vi "Test Client Timeout Returns Error.vi"(8 "error in (no error)":errorcluster) -> (0 "error out":errorcluster)   [LabVIEW 2019, in "RemoteControl.ZMQ.Tests.lvclass"]
uses:
  RemoteControl.ZMQ.Tests.lvclass
  C:/Program Files/National Instruments/LabVIEW 2019/user.lib/LevyLab/RemoteControl/RemoteControl/RemoteControl.lvclass
  <userlib>/LevyLab/RemoteControl/RemoteControl/RemoteControl.lvclass/RemoteControl.ctl
  <vilib>/numeric/Random Number (Range) U64.vi
  <vilib>/numeric/sub_Random U32.vi
  <vilib>/addons/_JKI Toolkits/Caraya/classes/Assert/Assert True.vi
  <userlib>/LevyLab/RemoteControl/RemoteControl/RemoteControl.lvclass
  <vilib>/addons/_JKI Toolkits/Caraya/classes/Assert/Assert.lvclass
  <vilib>/addons/_JKI Toolkits/Caraya/classes/Test/Test.lvclass
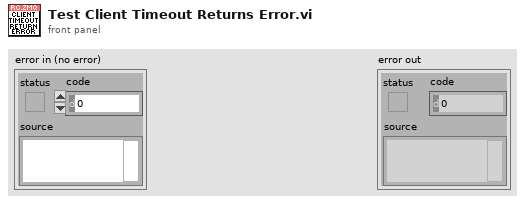
[diagram p1: front panel]
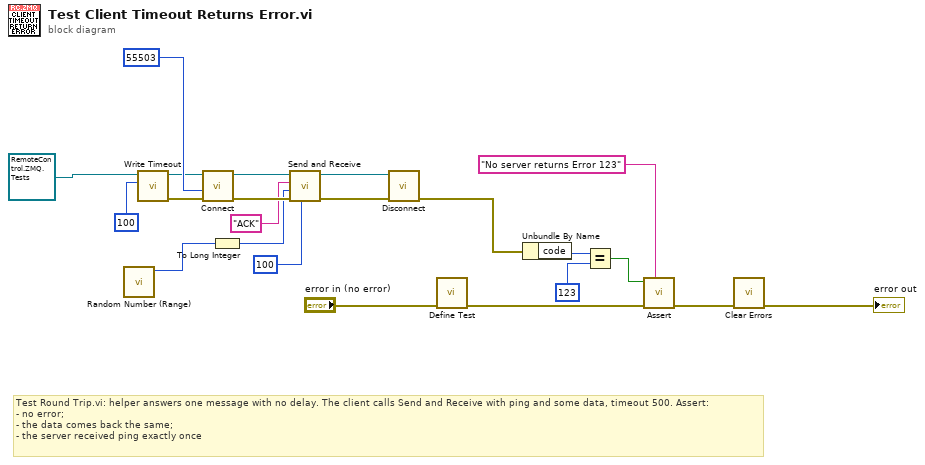
[diagram p0: block diagram]
diagram:
  # "Test Round Trip.vi: helper answers one message with no delay. The client calls Send and Receive with ping and some data, timeout 500. Assert:\n- no error;\n- the data comes back the same;\n- the server received ping exactly once"
  n1 = call-poly <vilib>:"Random Number (Range).vi"() -> ("number"=w15:u64)  [unwired: 11 in]
  n2 = call <userlib>:"Write Timeout.vi"("timeout (ms) [500]"=100 ("timeout in ms (100)"), "RemoteControl in"=refnum<class "RemoteControl.ZMQ.Tests.lvclass"> refnum ("RemoteControl.ZMQ.Tests.lvclass")) -> ("error out"=w13:errorcluster, "RemoteControl out"=w12:refnum<class "RemoteControl.ZMQ.Tests.lvclass">)  [unwired: 8 in]
  n3 = call <userlib>:"Connect.vi"("error in (no error)"=w13, "Port"=u16 55503, "RemoteControl in"=w12) -> ("error out"=w20:errorcluster, "RemoteControl out"=w22:refnum<class "RemoteControl.ZMQ.Tests.lvclass">)  [unwired: 7 in]
  n4 = To Long Integer(number=w15) -> (32bit integer=w10:i32)
  n5 = call <userlib>:"Send and Receive.vi"("timeout (ms) [500]"=100, "error in (no error)"=w20, "Data"=w10, "Command"="ACK", "RemoteControl in"=w22) -> ("error out"=w19:errorcluster, "RemoteControl out"=w21:refnum<class "RemoteControl.ZMQ.Tests.lvclass">)  [unwired: 3 in, 2 out]
  n6 = call <userlib>:"Disconnect.vi"("error in (no error)"=w19, "RemoteControl in"=w21) -> ("error out"=w4:errorcluster)  [unwired: 8 in, 1 out]
  n7 = call <vilib>:"Define Test.vi"("error in (no error)"="error in (no error)") -> ("error out"=w8:errorcluster)  [unwired: 9 in, 1 out]
  n8 = Unbundle By Name(w4) -> ("code"=w6:i32)
  n9 = Equal?(x=w6, y=123 ("error code (1)")) -> (x = y?=w3:bool)
  n10 = call-poly <vilib>:"Assert.vi"("Label"="No server returns Error 123", "error in (no error)"=w8, "True?"=w3) -> ("error out"=w16:errorcluster)  [unwired: 7 in, 1 out]
  n11 = call <vilib>:"Clear Errors.vi"("error in (no error)"=w16) -> ("error out"=→"error out":errorcluster)  [unwired: 5 in, 1 out]
